vi "OwnCompat20261012_Native_Create.vi"() -> ()   [LabVIEW 2024]
panel:
  out "error out":errorcluster caption="错误输出"
  in  "output_path":path
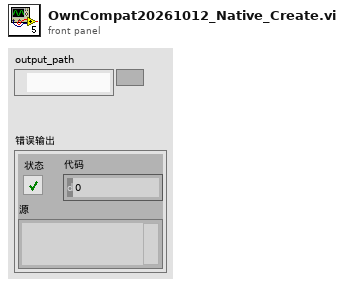
[diagram p1: front panel]
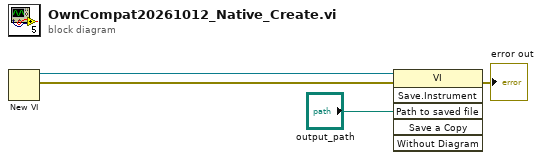
[diagram p0: block diagram]
diagram:
  n1 = New VI ("新建VI")() -> (0:w3:errorcluster, 3:w4:refnum<vi>)  [unwired: 7 in]
  n2 = invoke class="VI" method="Save.Instrument"(reference=w4, error in=w3, "Path to saved file"="output_path") -> (error out=→"error out":errorcluster)  [unwired: 3 in, 5 out]
